vi "Judgment_based_storage.vi"(10 "日志内容":string[](array[string]), 11 "日志名":string[](array[string])) -> (2 "新日志数组":string[](array[string]))   [LabVIEW 2018, in "Log_class.lvlib"]
uses:
  Log_class.lvlib
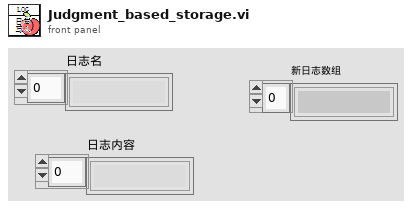
[diagram p1: front panel]
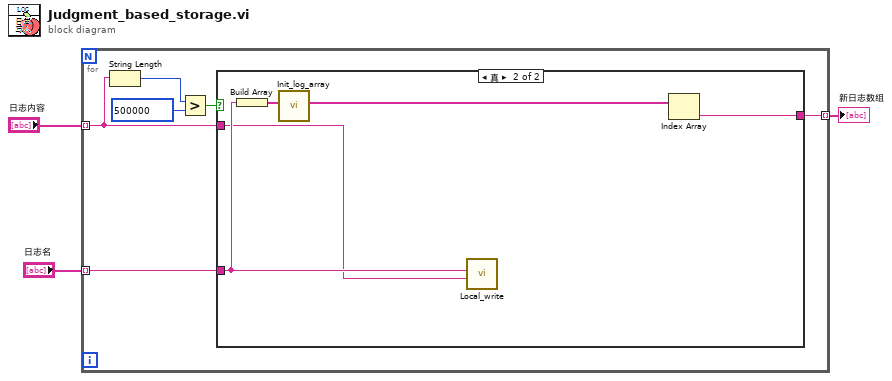
[diagram p0: block diagram]
diagram:
  n1 = for {
    tunnel: "日志内容" -> [w6] mode=indexing
    tunnel: "日志名" -> [w5] mode=indexing
    tunnel: [w4] -> w1 mode=indexing
    n2 = String Length(string=w6) -> (length=w9:i32)
    n3 = Greater?(x=w9, y=500000) -> (0:w7:bool)
    n4 = case shown="真" w7 {
      tunnel: w6 -> [w10 w11]
      tunnel: [w10 w13] -> w4
      tunnel: w5 -> [_ w12]
      frame False {
      }
      frame True {
        n5 = Build Array(w12) -> (w15:string[])
        n6 = call "Init_log_array.vi"("要创建的日志名字"=w15) -> ("数组"=w14:string[])  [unwired: 10 in]
        n7 = call "Local_write.vi"("内容"=w11, "名字"=w12) -> ()  [unwired: 9 in, 1 out]
        n8 = Index Array(array=w14) -> (element=w13:string)  [unwired: 1 in]
      }
    }
  }
  "新日志数组" <- w1
